vi "testParseStateQueueError.vi"(8 "error in (no error)":errorcluster, 11 "testStateMachineUtilities in":refnum<class "testStateMachineUtilities.lvclass">) -> (0 "error out":errorcluster, 3 "testStateMachineUtilities out":refnum<class "testStateMachineUtilities.lvclass">)   [LabVIEW 2020, in "testStateMachineUtilities.lvclass"]
uses:
  testStateMachineUtilities.lvclass
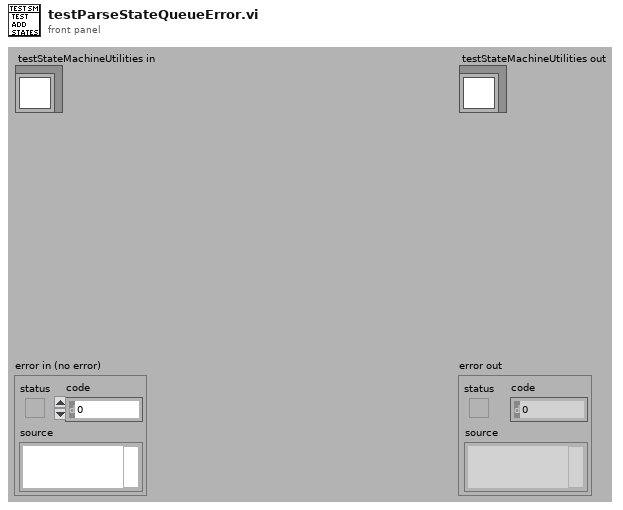
[diagram p1: front panel]
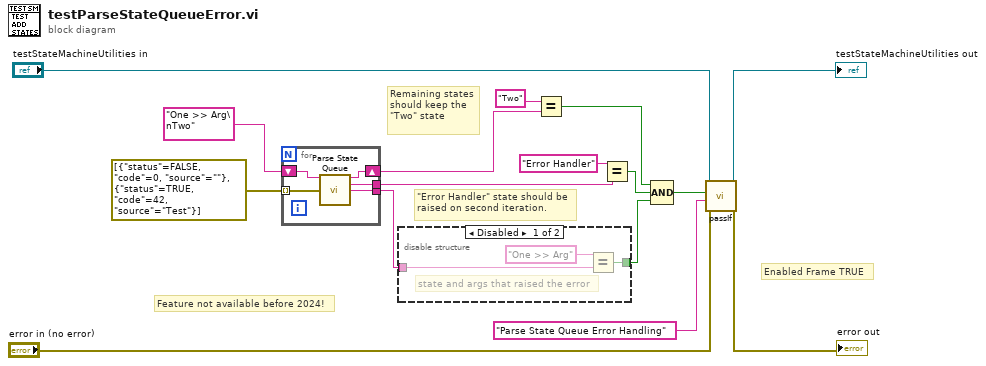
[diagram p0: block diagram]
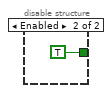
[diagram p2: hidden frame]
diagram:
  # "Enabled Frame TRUE"
  # "Feature not available before 2024!"
  # "\"Error Handler\" state should be raised on second iteration."
  # "Remaining states should keep the \"Two\" state"
  n1 = for {
    tunnel: errorcluster[] [{"status"=FALSE, "code"=0, "source"=""}, {"status"=TRUE, "code"=42, "source"="Test"}] -> [w21] mode=indexing
    tunnel: [w19] -> w3
    tunnel: [w18] -> w10
    shift-right: [w17] -> w5
    shift-left: "One >> Arg\nTwo" ("State Queue") -> [w20]
    n2 = call "Parse State Queue.vi"("State Queue"=w20, "Error In (no error)"=w21) -> ("Remaining States"=w17:string, "Current State"=w18:string, "Arguments"=w19:string)  [unwired: 11 in]
  }
  n3 = disable-structure shown="Disabled" {
    disable-tunnel: w3 -> [w23 _]
    disable-tunnel: [w22 TRUE] -> w2
    frame Disabled {
      # "state and args that raised the error"
      n4 = Equal?(x="One >> Arg", y=w23) -> (x = y?=w22:bool)
    }
    frame Enabled {
    }
  }
  n5 = Equal?(x="Two" ("State Queue"), y=w5) -> (x = y?=w1:bool)
  n6 = Equal?(x="Error Handler", y=w10) -> (x = y?=w9:bool)
  n7 = Compound Arithmetic op=AND(w1, w9, w2) -> (w8:bool)
  n8 = call-dynamic "passIf.vi"("error in (no error)"="error in (no error)", "message (\"\")"="Parse State Queue Error Handling", "pass"=w8, "TestCase in"="testStateMachineUtilities in") -> ("error out"=→"error out":errorcluster, "TestCase out"=→"testStateMachineUtilities out":refnum<class "testStateMachineUtilities.lvclass">)  [unwired: 6 in]
